vi "writeUserModePref.vi"(5 "value to write":string, 11 "error in":errorcluster) -> (4 "found?":bool, 15 "error out":errorcluster)   [LabVIEW 2023]
uses:
  <vilib>/Utility/config.llb/Write Key (String).vi
  <vilib>/Utility/config.llb/NI_LVConfig.lvlib
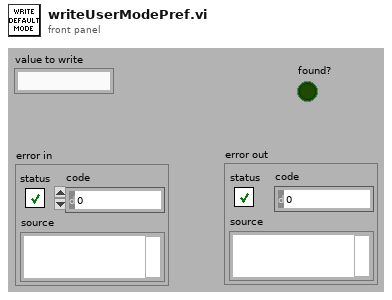
[diagram p1: front panel]
types:
  T1 = typedef "NI_LVConfig.lvlib/Config Data RefNum.ctl" = refnum<k1>
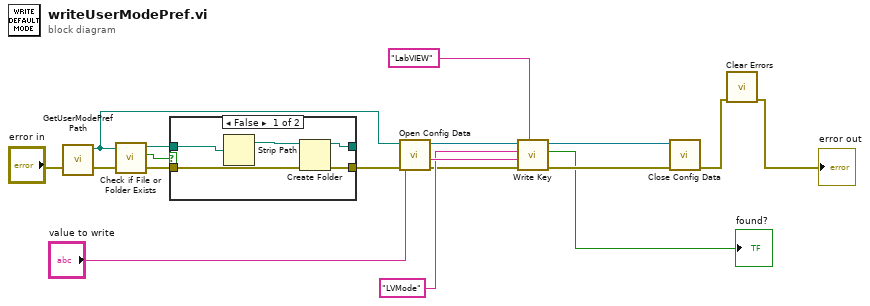
[diagram p0: block diagram]
diagram:
  n1 = call <resource>:"GetUserModePrefPath.vi"() -> ("prefpath"=w3:path)  [unwired: 11 in]
  n2 = call <vilib>:"Check if File or Folder Exists.vi"("error in (no error)"="error in", "path"=w3) -> ("error out"=w5:errorcluster, "file or folder exists?"=w7:bool, "dup path"=w6:path)  [unwired: 7 in]
  n3 = case shown="False" w7 {
    tunnel: w6 -> [w18 w23]
    tunnel: [w19 w23] -> _
    tunnel: w5 -> [w21 w22]
    tunnel: [w20 w22] -> w4
    frame False {
      n4 = Strip Path(path=w18) -> (stripped path=w17:path)  [unwired: 1 out]
      n5 = Create Folder(path (use dialog)=w17, error in=w21) -> (created path=w19:path, error out=w20:errorcluster)  [unwired: 1 in, 1 out]
    }
    frame True {
    }
  }
  n6 = call <vilib>:"Open Config Data.vi"("error in (no error)"=w4, "configuration file path"=w3) -> ("error out"=w10:errorcluster, "refnum"=w11:T1)  [unwired: 7 in, 1 out]
  n7 = call-poly <vilib>:"Write Key.vi"("section"="LabVIEW", "error in (no error)"=w10, "value"="value to write", "key"="LVMode", "refnum"=w11) -> ("error out"=w16:errorcluster, "found?"=→"found?":bool, "refnum out"=w15:T1)  [unwired: 4 in]
  n8 = call <vilib>:"Close Config Data.vi"("error in (no error)"=w16, "refnum"=w15) -> ("error out"=w2:errorcluster)  [unwired: 8 in, 1 out]
  n9 = call <vilib>:"Clear Errors.vi"("error in (no error)"=w2) -> ("error out"=→"error out":errorcluster)  [unwired: 5 in, 1 out]
